vi "AI Base Globals.vi"() -> ()   [LabVIEW 2023, in "LabVIEW AI Base.lvlib"]
uses:
  LabVIEW AI Base.lvlib
  <vilib>/httpClient/ClientHandle.ctl
  <vilib>/httpClient/LabVIEWHTTPClient.lvlib
panel:
  in  "Tab Control":enum32{"Python Settings", "LLM Settings"}(tab)=enum."LLM Settings"
  out "Python Session":refnum<k35>
  in  "venv path":path=path "C:/dev/labview-ai"
  in  "Anaconda path":path=path "C:/ProgramData/miniforge3"
  in  "Python version":string="3.10"
  in  "conda env name":string="ai"
  out "Http Client Handle":T1
  in  "OpenAI API URL":string="http://localhost:1234/v1" caption="OpenAI API URL (e.g. OpenRouter, LM Studio)"
  in  "API Key":string
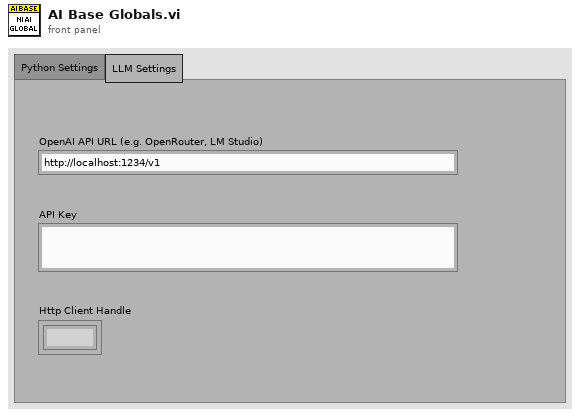
[diagram p1: front panel]
types:
  T1 = typedef "LabVIEWHTTPClient.lvlib/ClientHandle.ctl" = refnum<k1>
diagram:
